vi "湿度测量 - HM1.vi"(7 "CSM Name":string="HM1") -> ()   [LabVIEW 2026, in "UI-湿度测量.lvlib"]
uses:
  Supports/Sample Settings.ctl
  Data ColndSave/Supports/Time and Data.ctl
  <userlib>/_NEVSTOP/Communicable State Machine(CSM)/_Polymophic/CSM - Filter Duplicated Lines.vi
  a3283b4f-3d7d-475f-8286-b95f18be6a9d.vi
  adb26933-f597-44e1-90e5-85e3d61c535a.vi
  c6692627-02fb-4556-9c5d-59e6097d0856.vi
  8c0fc226-3871-4866-9b38-f175316b3ef9.vi
  8417ea6c-3bd9-4cd5-8933-b29b0935beb3.vi
  c0a7cae7-a94b-4088-a6e9-4f476a10c4ba.vi
  <userlib>/_NEVSTOP/Communicable State Machine(CSM)/_Polymophic/CSM - Replace Marks in Messages.vi
  5163a33a-69e0-492d-a74e-a390bdb1a610.vi
  afa19ee1-f3d3-482d-9a92-e9809811bd36.vi
  6c4ca8cd-bc2b-4d91-b813-4304b5b94d16.vi
  <userlib>/_NEVSTOP/Communicable State Machine(CSM)/AdvanceAPI/CSM - Compact Multiple States.vi
  <userlib>/_NEVSTOP/Communicable State Machine(CSM)/AdvanceAPI/CSM - Break Down Multiple States String.vi
  <userlib>/_NEVSTOP/Communicable State Machine(CSM)/_Shared/Remove Comments from Single-line.vi
  <userlib>/_NEVSTOP/Communicable State Machine(CSM)/_Shared/Split Single-line Message.vi
  <userlib>/_NEVSTOP/Communicable State Machine(CSM)/_Shared/Trim Single-line Text.vi
  <userlib>/_NEVSTOP/Communicable State Machine(CSM)/AdvanceAPI/CSM - Revert Arguments-Safe String.vi
  <userlib>/_NEVSTOP/Communicable State Machine(CSM)/AdvanceAPI/CSM - Make String Arguments Safe.vi
  c6692627-02fb-4556-9c5d-59e6097d0856.vi/99de0c97-112a-4c86-9094-c187659127e1.vi
  <userlib>/_NEVSTOP/Communicable State Machine(CSM)/Utility/Build Error Cluster.vi
  8417ea6c-3bd9-4cd5-8933-b29b0935beb3.vi/99de0c97-112a-4c86-9094-c187659127e1.vi
  <userlib>/_NEVSTOP/Communicable State Machine(CSM)/AdvanceAPI/CSM - Keywords.vi
  <userlib>/_NEVSTOP/Communicable State Machine(CSM)/addons/API-String-Arugments-Support/_Support/Data To API String Arguments.vi
  <userlib>/_NEVSTOP/Communicable State Machine(CSM)/addons/INI-Static-Variable-Support/_Support/instances/_CSM - Read File Logger Configuration - v1.0.vi
  <vilib>/Utility/Data Type/Get Type Information.vi
  <userlib>/_NEVSTOP/Communicable State Machine(CSM)/addons/API-String-Arugments-Support/_Support/Data To SingleElementsArray_csm.vi
  <userlib>/_NEVSTOP/Communicable State Machine(CSM)/addons/INI-Static-Variable-Support/_Support/Parse Used Session and Name.vi
  <userlib>/_NEVSTOP/Communicable State Machine(CSM)/addons/INI-Static-Variable-Support/_Support/INI-FGV(lvlibp).vi
  <userlib>/_NEVSTOP/Communicable State Machine(CSM)/addons/INI-Static-Variable-Support/_Support/Populate String with INI Variable.vi
  <userlib>/_NEVSTOP/Communicable State Machine(CSM)/addons/API-String-Arugments-Support/_Support/Convert API String Arguments to Data(variant).vi
  <userlib>/_NEVSTOP/Communicable State Machine(CSM)/addons/API-String-Arugments-Support/_Support/SingleElementsArray To Data_csm.vi
  <userlib>/_NEVSTOP/Communicable State Machine(CSM)/addons/MassData-Parameter/_support/FGV-MassData(lvlibp).vi
  <userlib>/_NEVSTOP/Communicable State Machine(CSM)/Communicable State Machine.lvlib
  Acquisition/Acquisition.lvlib
  <userlib>/_NEVSTOP/Communicable State Machine(CSM)/addons/MassData-Parameter/CSM MassData Parameter Support.lvlib
  <userlib>/_NEVSTOP/Communicable State Machine(CSM)/addons/INI-Static-Variable-Support/INI-Static-Variable-Support.lvlib
  <userlib>/_NEVSTOP/Communicable State Machine(CSM)/addons/Watchdog/CSM Watchdog.lvlib
  <userlib>/_NEVSTOP/Communicable State Machine(CSM)/addons/Logger/CSM File Logger.lvlib
  Logging/Logging.lvlib
  Data ColndSave/Data Collection and Save.lvlib
panel:
  in  "停止":bool
  in  "湿度显示":enum32{"温度采集", "Status"}(tab)
  in  "湿度采集开关":bool
  in  "USB Port":refnum<visa-resource-name>="COM3"
  in  "Interval(s)":dbl=0.5
  out "湿度":waveform(dbl)(graph)
  in  "子程序？":bool
  out "Error Occurred":errorcluster caption="温度采集-错误输出"
  out "State History":string
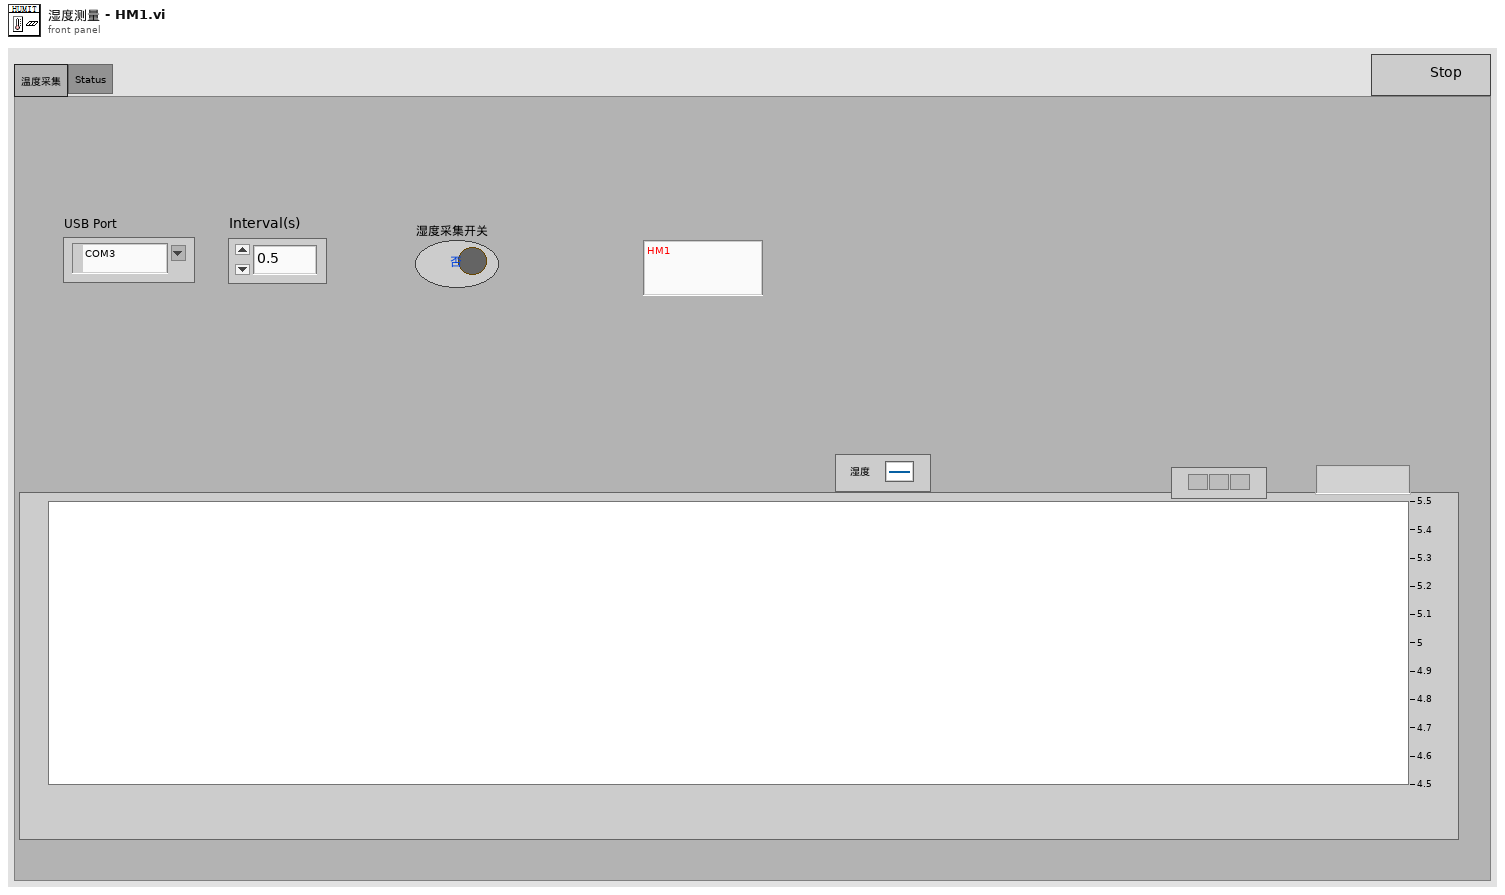
[diagram p1: front panel]
types:
  T1 = cluster{"Enable":bool, "Limit":cluster{"FileSize":i64, "FileNum":i32}, "Timestamp.Format":string, "AutoExit":bool}
  T2 = enum32{"Invalid", "Standard", "Closed", "Hidden", "Minimized", "Maximized"}
  T3 = enum32{"invalid app kind", "Development System", "Run Time System", "Student Edition", "Embedded LabVIEW", "Evaluation", "Custom"}
  T4 = typedef "Communicable State Machine.lvlib/_CSM_Response Source Message.ctl" = cluster{"‘State":string, "’Arguments":string, "’Error":errorcluster}
  T5 = cluster{"Current VI Reference":refnum<vi>, "Close Panel on Exit?":bool}
  T6 = typedef "UI-湿度测量.lvlib/Sample Settings.ctl" = cluster{"USB Port":refnum<visa-resource-name>, "Interval(s)":dbl}
  T7 = typedef "Data Collection and Save.lvlib/Time and Data.ctl" = cluster{"采集时间":timestamp, "Data":dbl[]}
  T8 = cluster{"Core":cluster{"Current VI Reference":refnum<vi>, "Close Panel on Exit?":bool}, "Sample Settings":T6, "Time and Data":T7, "子程序？":bool}
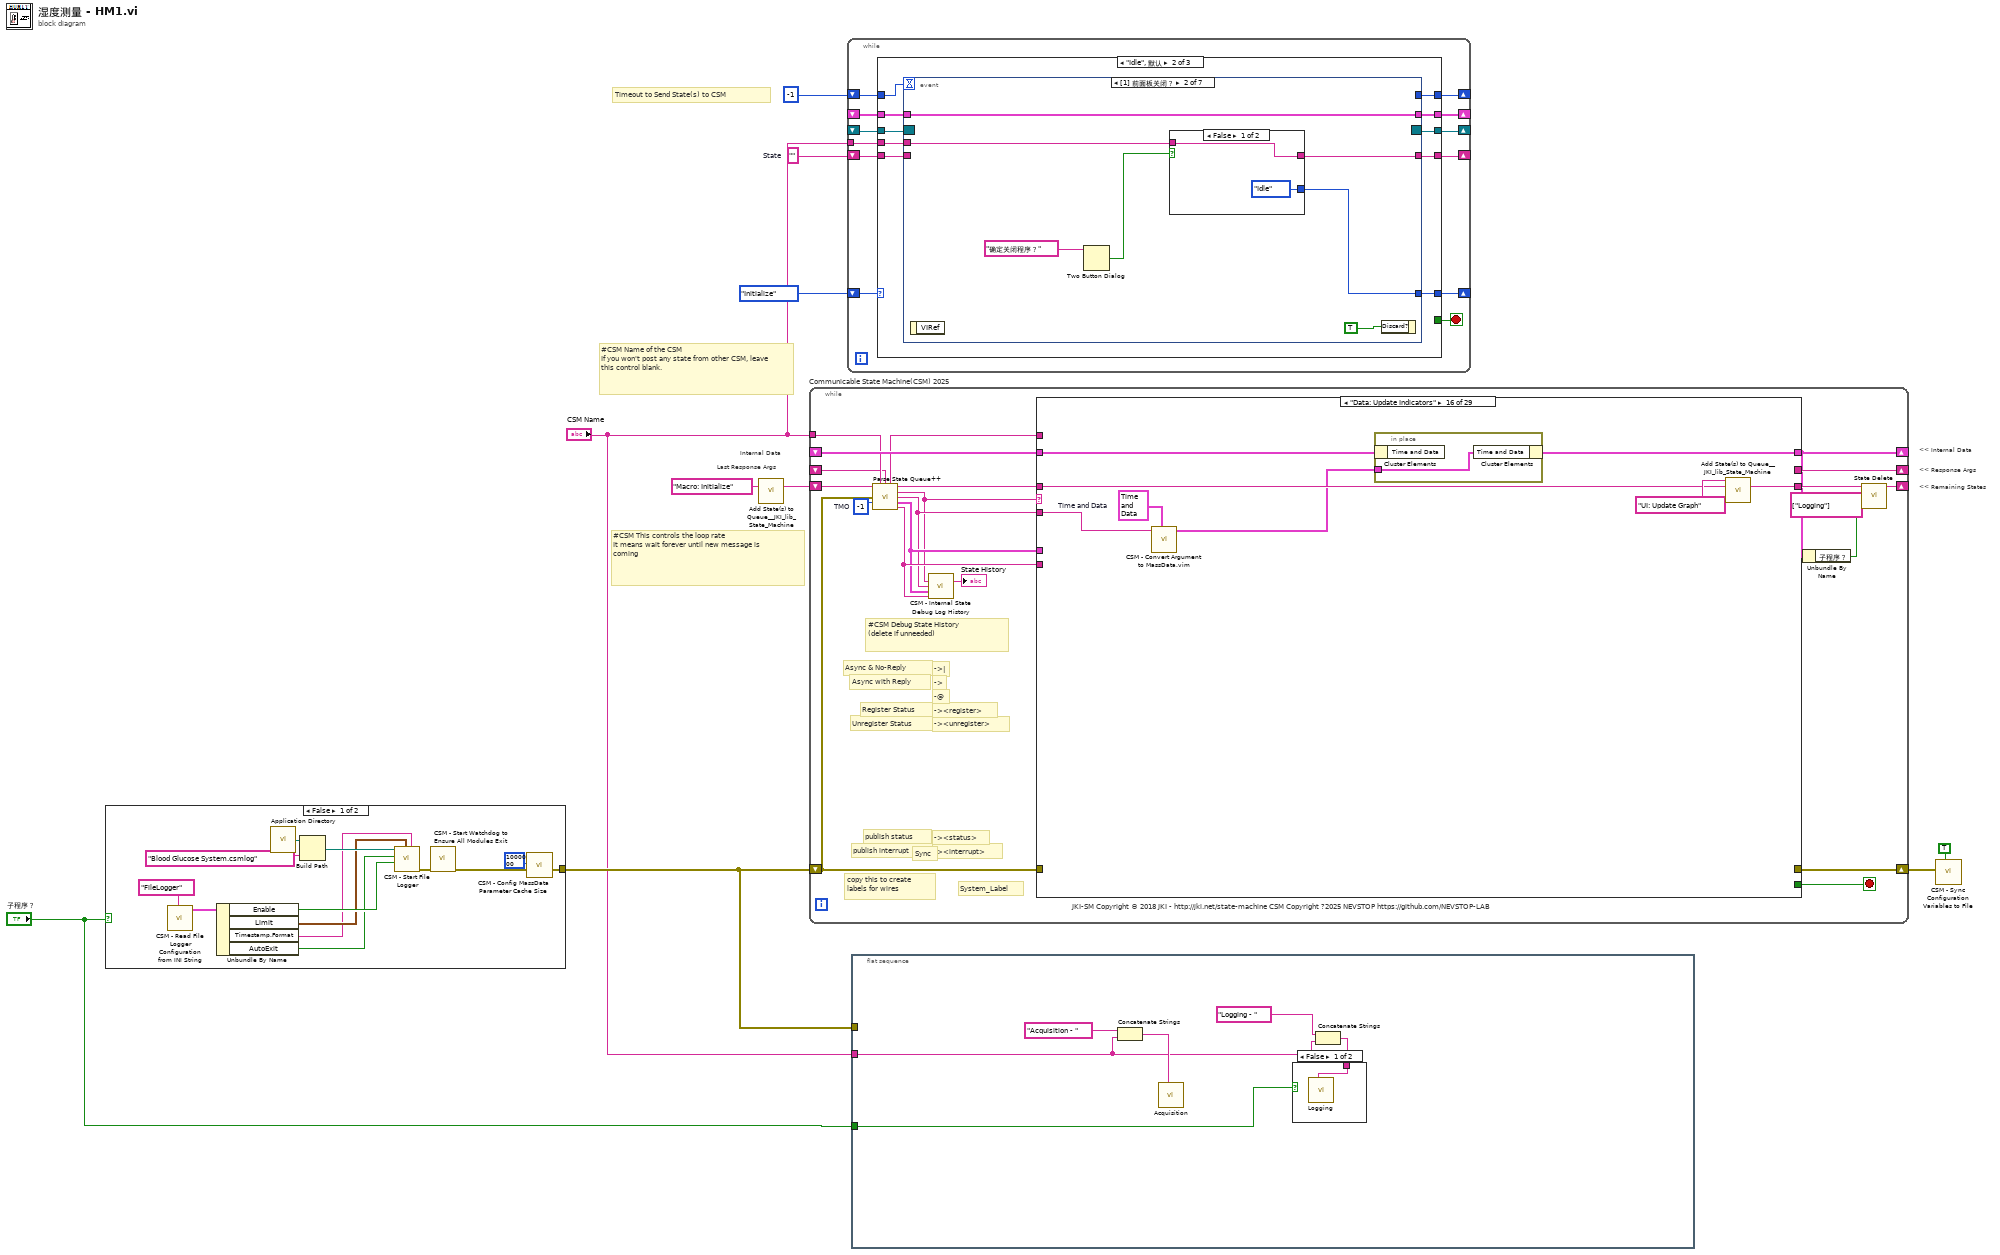
[diagram p0: block diagram]
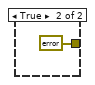
[diagram p2: hidden frame]
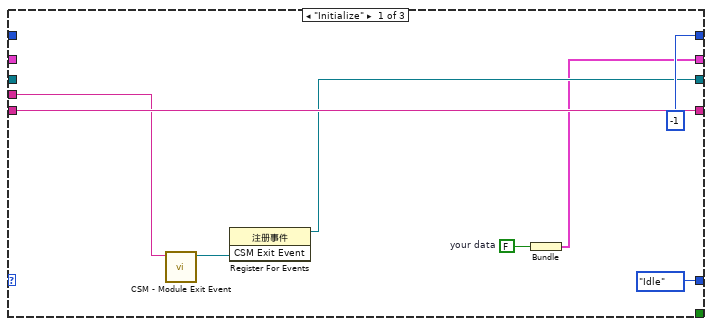
[diagram p4: hidden frame]
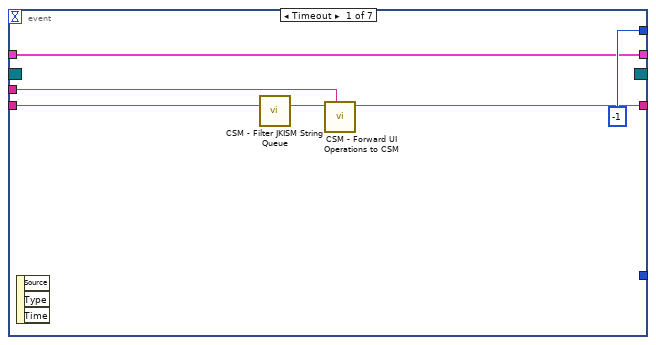
[diagram p5: hidden frame]
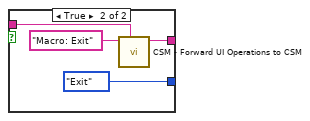
[diagram p6: hidden frame]
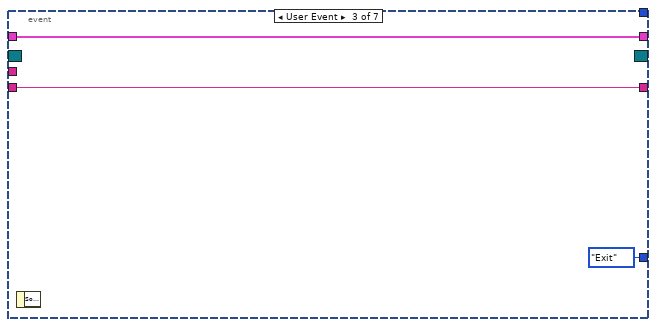
[diagram p7: hidden frame]
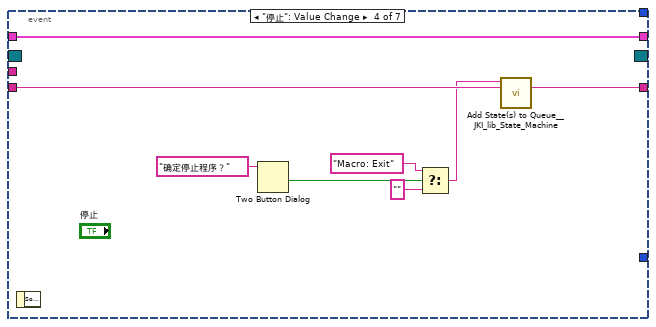
[diagram p8: hidden frame]
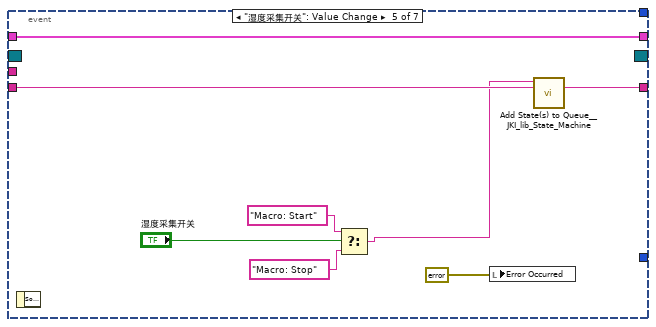
[diagram p9: hidden frame]
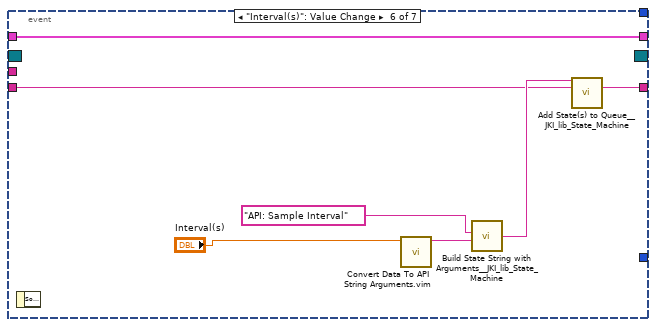
[diagram p10: hidden frame]
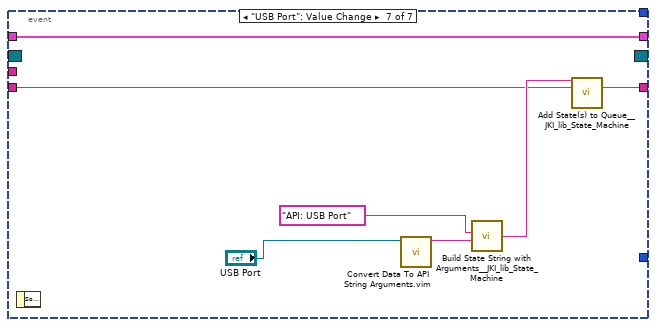
[diagram p11: hidden frame]
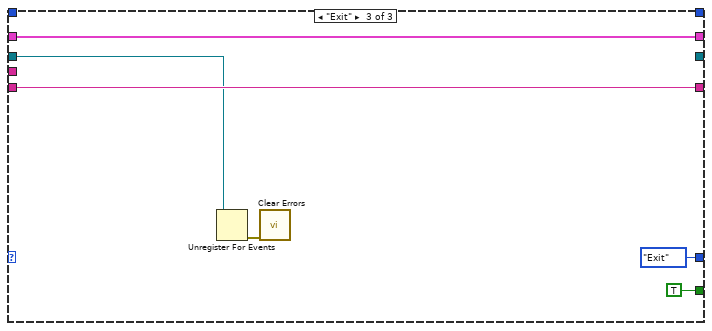
[diagram p12: hidden frame]
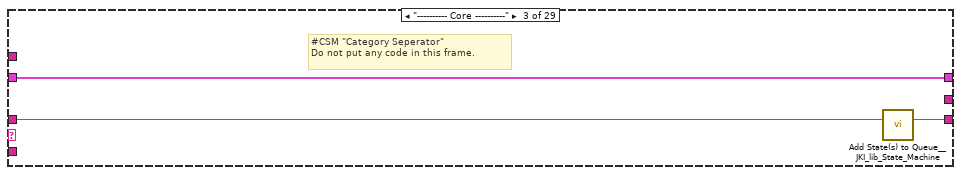
[diagram p15: hidden frame]
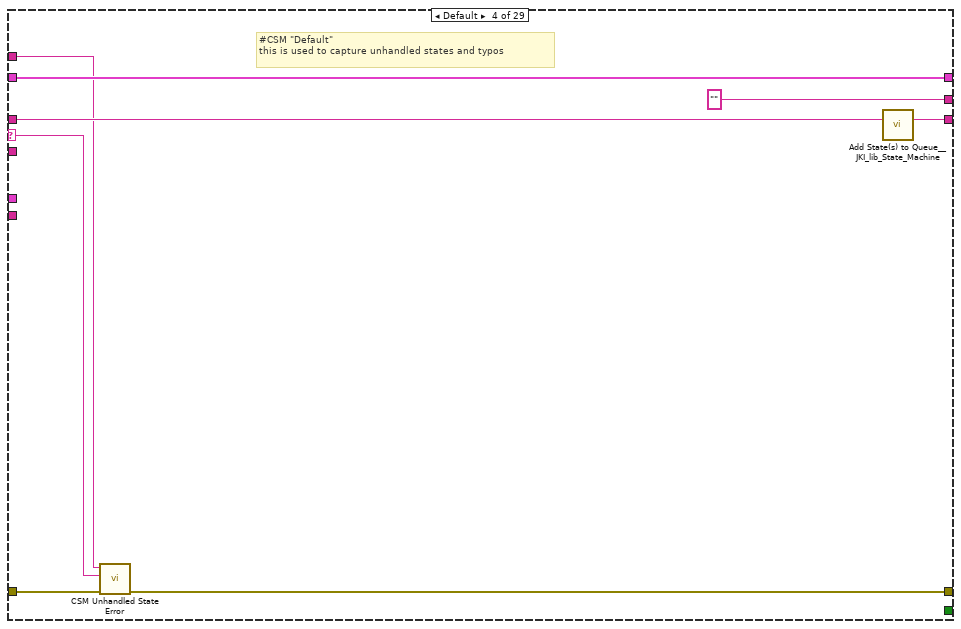
[diagram p16: hidden frame]
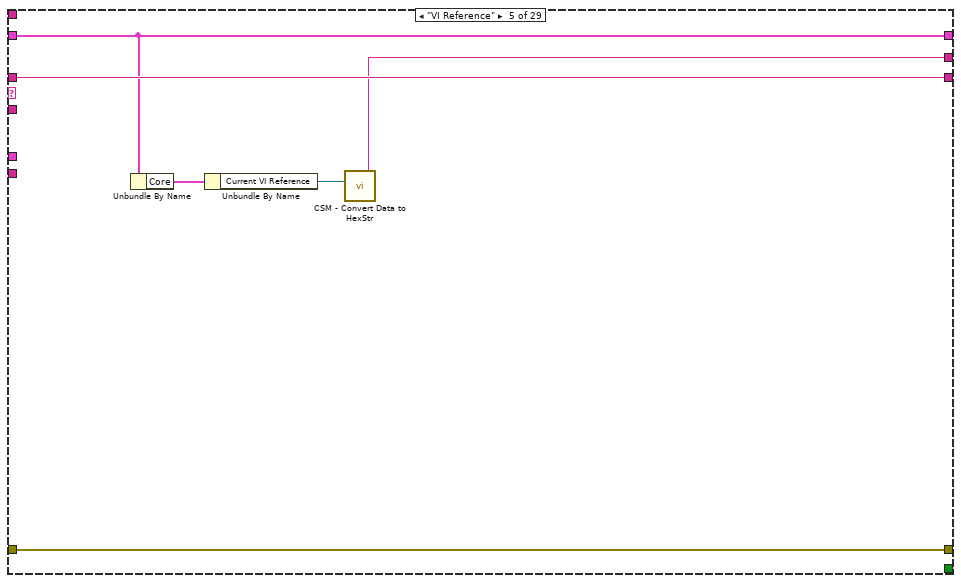
[diagram p17: hidden frame]
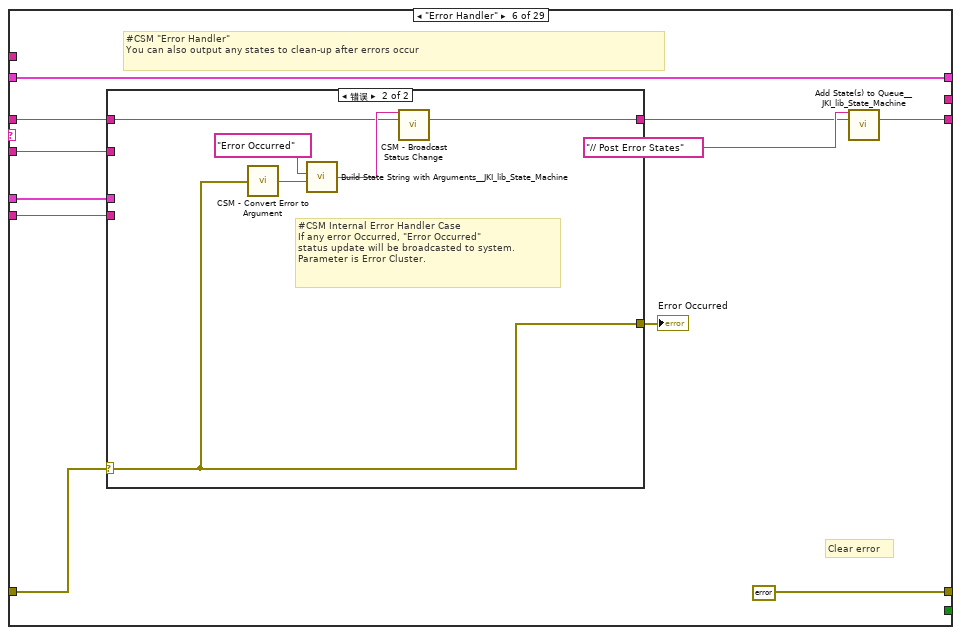
[diagram p18: hidden frame]
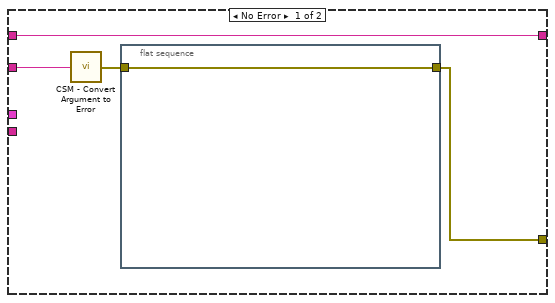
[diagram p19: hidden frame]
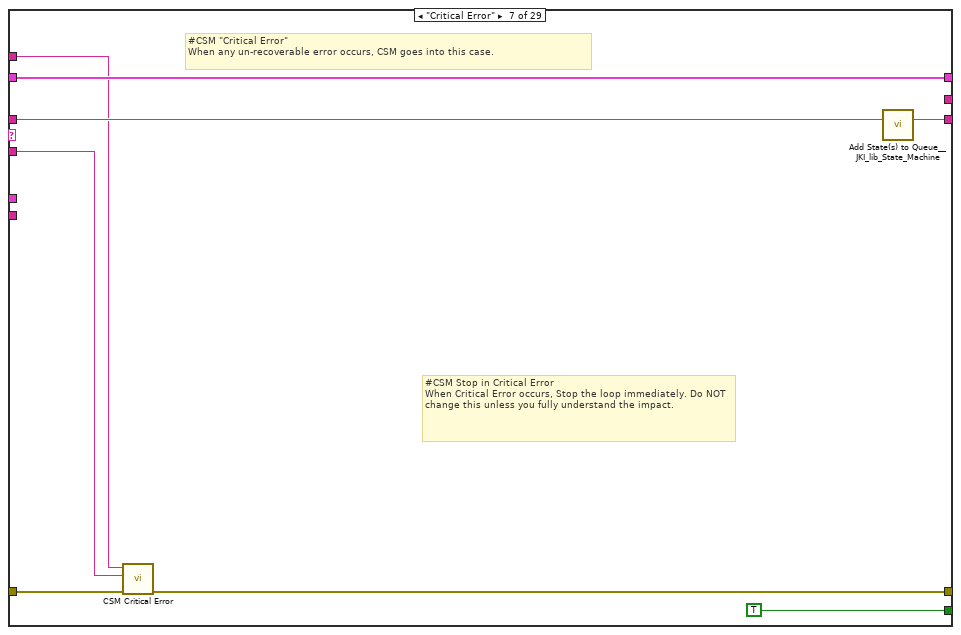
[diagram p20: hidden frame]
diagram:
  w9 = ""  # State
  # "Timeout to Send State(s) to CSM"
  # "Last Response Args"
  # "Internal Data"
  # "#CSM Name of the CSM\nIf you won't post any state from other CSM, leave this control blank."
  # "#CSM This controls the loop rate\nIt means wait forever until new message is coming"
  # "<< Internal Data"
  # "<< Response Args"
  # "<< Remaining States"
  n1 = case shown="False" "子程序？" {
    tunnel: [w11 errorcluster {"status"=FALSE, "code"=0, "source"=""} ("Error out")] -> w5
    frame False {
      n2 = call-poly <userlib>:"CSM - Read File Logger Configuration from INI String.vi"("Section Name(\"FileLogger\")"="FileLogger" ("Section Name(\"\" as Default)")) -> ("FileLogger Configuration-v1"=w18:T1)  [unwired: 7 in, 1 out]
      n3 = Unbundle By Name(w18) -> ("Enable"=w17:bool, "Limit"=w16:cluster{"FileSize":i64, "FileNum":i32}, "Timestamp.Format"=w14:string, "AutoExit"=w15:bool)
      n4 = call <vilib>:"Application Directory.vi"() -> ("Application Directory"=w23:path)
      n5 = Build Path(base path=w23, name or relative path="Blood Glucose System.csmlog") -> (appended path=w21:path)
      n6 = call <userlib>:"CSM - Start File Logger.vi"("Timestamp Format"=w14, "Log Limit"=w16, "Watchdog? (T)"=w17, "Exit When All Module Exist? (F)"=w15, "Log File Path"=w21) -> ("error out"=w20:errorcluster)  [unwired: 4 in, 2 out]
      n7 = call <userlib>:"CSM - Start Watchdog to Ensure All Modules Exit.vi"("error in (no error)"=w20) -> ("error out"=w12:errorcluster)  [unwired: 10 in]
      n8 = call <userlib>:"CSM - Config MassData Parameter Cache Size.vi"("Error in"=w12, "Size (50M)"=1000000 ("size(1M)")) -> ("Error out"=w11:errorcluster)  [unwired: 9 in]
    }
    frame True {
    }
  }
  n9 = call <vilib>:"Add State(s) to Queue__JKI_lib_State_Machine.vi"("State(s) in (\"\")"="Macro: Initialize" ("Init State(\"Macro: Initialize\")")) -> ("States Out"=w6:string)  [unwired: 14 in]
  n10 = while "Communicable State Machine(CSM) 2025" {
    shift-right: [w26] -> _
    shift-left: _ -> [w41]
    shift-right: [w43] -> w3
    shift-left: w5 -> [w31]
    shift-right: [w28] -> _
    shift-left: w6 -> [w44]
    tunnel: "CSM Name" -> [w38]
    shift-right: [w39] -> _
    shift-left: _ -> [w33]
    stop <- w42 stop-if-true
    w40 = -1  # TMO
    # "#CSM Debug State History\n(delete if unneeded)"
    # "-><interrupt>"
    # "-><status>"
    # "-><unregister>"
    # "-><register>"
    # "-@"
    # "->"
    # "->|"
    # "publish interrupt"
    # "publish status"
    # "Unregister Status"
    # "Register Status"
    # "Sync"
    # "Async with Reply"
    # "Async & No-Reply"
    # "JKI-SM Copyright © 2018 JKI - http://jki.net/state-machine CSM Copyright ?2025 NEVSTOP https://github.com/NEVSTOP-LAB"
    # "copy this to create labels for wires"
    # "System_Label"
    n11 = call <userlib>:"Parse State Queue++.vi"("State Queue"=w44, "Name (\"\" to Use UUID)"=w38, "Response Arguments"=w33, "Previous Error"=w31, "Dequeue (1 ms)"=w40) -> ("Name Used"=w32:string, "Remaining States"=w45:string, "Current State"=w34:string, "Arguments"=w35:string, "Additional Information"=w36:T4, "Source CSM"=w37:string)  [unwired: 5 in]
    n12 = call <userlib>:"CSM - Internal State Debug Log History.vi"("State"=w34, "Arguments (\"\")"=w35, ">> Response Source Message >>"=w36, "Source (\"\")"=w37) -> ("Debug Log"=→"State History":string)  [unwired: 11 in]
    n13 = case shown="\"Data: Update Indicators\"" w34 {
      selector: w34 -> [_ _ _ w56 _ _ _ _ _ _ _ _ _ _ _ _ _ _ _ _ _ _ _ _ _ _ _ _ _]
      tunnel: w45 -> [w46 w49 w52 w60 w65 w71 w96 w102 w108 w118 w125 w137 w141 w144 w157 w164 w175 w178 w186 w197 w203 w208 w214 w224 w231 w237 w240 w251 w258]
      tunnel: w35 -> [_ _ _ _ _ w70 w92 w99 w105 w112 _ _ _ _ _ w162 _ _ _ _ w199 _ _ _ _ _ _ w245 w256]
      tunnel: w41 -> [w47 w48 w50 w58 w64 w76 w94 w100 w106 w116 w124 w131 w139 w142 _ w160 w170 w176 w179 w195 w201 w206 w212 w221 w229 w235 w242 w244 w255]
      tunnel: [_ _ _ w53 w66 errorcluster {"status"=FALSE, "code"=0, "source"=""} ("error out") w89 w97 w103 w119 _ _ _ _ _ _ w171 _ _ _ _ _ _ _ _ _ _ _ _] -> w43
      tunnel: w31 -> [_ _ _ w54 w66 w74 w90 w98 w104 _ _ _ _ _ _ _ w172 _ _ _ _ _ _ _ _ _ _ _ _]
      tunnel: [w46 w49 w51 w59 w65 w72 w95 w101 w107 w117 w125 w136 w140 w143 w156 w163 w174 w177 w185 w196 w202 w207 w213 w223 w230 w236 w241 w252 w259] -> w29
      tunnel: [_ _ _ _ _ _ TRUE _ _ _ _ _ TRUE _ _ _ _ _ _ _ _ _ _ _ _ _ _ _ _] -> w42
      tunnel: [w47 w48 w50 w58 w64 w76 w94 w100 w106 w115 w124 w135 w139 w142 w155 w159 w170 w176 w179 w195 w201 w206 w212 w220 w229 w235 w242 w243 w254] -> w26
      tunnel: w37 -> [_ _ _ _ _ w69 _ _ _ w113 _ _ _ _ _ _ _ _ _ _ _ _ _ _ _ _ _ _ _]
      tunnel: w36 -> [_ _ _ _ _ w68 _ _ _ w114 _ _ _ _ _ _ _ _ _ _ _ _ _ _ _ _ _ _ _]
      tunnel: [_ _ _ "" w61 _ _ _ _ _ _ _ _ _ _ _ _ _ _ _ _ _ _ _ _ _ _ _ _] -> w39
      tunnel: w32 -> [_ _ _ w55 _ _ w91 _ _ _ _ _ _ _ w151 _ w167 _ _ _ _ _ w210 w217 w227 w233 _ w249 _]
      frame "", "Idle" {
        # "#CSM \"Idle/Event Handler\"\nexecutes when the state queue is empty"
      }
      frame "CSM Documentation" {
        # "#CSM State Syntax\n\n// Comment line, all text to the right of “//” will be ignored\n// Local Message Example\nDoSth: DoA >> Arguments\n\n// Sync Call Example\nAPI: xxxx >> Arguments -@ TargetModule\n\n// Async Call Example\nAPI: xxxx >> Arguments -> TargetModule\n\n// Async Call without Reply Example\nAPI: xxxx >> Arguments ->| TargetModule\n\n// Broadcast normal status:\nStatus >> StatusArguments  -><status>\n\n// Broadcast Interrupt status:\nInterrupt >> StatusArguments  -><interrupt>\n\n// Register Source Module's status to Handler Module\nStatus@Source Module >> Handler Module@Handler Module -><register>\n\n// Unegister Source Module's status\nStatus@Source Module >> Handler Module -><unregister>"
        # "#CSM README FIRST\n\nCommunicable State Machine(CSM) is a LabVIEW application framework that builds upon JKI State Machine(JKISM). It follows the pattern of JKISM and extends the keywords to describe message communication between modules, including concepts such as Sync-Message, Async-Message, Subscription/Unsubscription of status - essential elements for creating reusable code modules. For more information, please visit the CSM wiki: https://nevstop-lab.github.io/CSM-Wiki/\n\nFor instructions on JKI State Machine, visit: \n    http://jki.net/state-machine/\nFor information about CSM, visit: \n    https://github.com/NEVSTOP-LAB"
        # "#CSM \"Documentation\"\nCase for holding CSM Documenation"
      }
      frame "---------- Core ----------" {
        # "#CSM \"Category Seperator\"\nDo not put any code in this frame."
        n14 = call <vilib>:"Add State(s) to Queue__JKI_lib_State_Machine.vi"("State(s) in (\"\")"=w52) -> ("States Out"=w51:string)  [unwired: 14 in]
      }
      frame Default {
        # "#CSM \"Default\"\nthis is used to capture unhandled states and typos"
        n15 = call <userlib>:"CSM Unhandled State Error.vi"("error in (no error)"=w54, "Undefined State"=w56, "CSM Name"=w55) -> ("error out"=w53:errorcluster)  [unwired: 8 in]
        n16 = call <vilib>:"Add State(s) to Queue__JKI_lib_State_Machine.vi"("State(s) in (\"\")"=w60) -> ("States Out"=w59:string)  [unwired: 14 in]
      }
      frame "VI Reference" {
        n17 = Unbundle By Name(w64) -> ("Core"=w63:T5)
        n18 = Unbundle By Name(w63) -> ("Current VI Reference"=w62:refnum<vi>)
        n19 = call <userlib>:"CSM - Convert Data to HexStr.vi"("Variant"=w62) -> ("HEX String (0-9,A-F)"=w61:string)  [unwired: 8 in]
      }
      frame "Error Handler" {
        # "#CSM \"Error Handler\"\nYou can also output any states to clean-up after errors occur"
        # "Clear error"
        n20 = case shown="错误" w74 {
          selector: w74 -> [_ w83]
          tunnel: [w81 w85] -> w73
          tunnel: w71 -> [w81 w84]
          tunnel: w70 -> [w80 _]
          tunnel: w69 -> [_ _]
          tunnel: w68 -> [_ _]
          tunnel: [w78 w83] -> w67
          frame No Error {
            n21 = call <userlib>:"CSM - Convert Argument to Error.vi"("Argument"=w80) -> ("Error"=w79:errorcluster)  [unwired: 4 in]
            n22 = flat-sequence {
              tunnel: w79 -> [w82]
              tunnel: [w82] -> w78
              frame #0 {
              }
            }
          }
          frame Error {
            # "#CSM Internal Error Handler Case \nIf any error Occurred, \"Error Occurred\" \nstatus update will be broadcasted to system.\nParameter is Error Cluster."
            n23 = call <userlib>:"CSM - Convert Error to Argument.vi"("Error"=w83) -> ("Argument"=w87:string)  [unwired: 4 in]
            n24 = call <vilib>:"Build State String with Arguments__JKI_lib_State_Machine.vi"("Arguments (\"\")"=w87, "State"="Error Occurred" ("Status with Arguments")) -> ("State with Arguments"=w86:string)  [unwired: 4 in]
            n25 = call <userlib>:"CSM - Broadcast Status Change.vi"("Status With Arguments"=w86, "State Queue"=w84) -> ("Remaining States"=w85:string)  [unwired: 13 in]
          }
        }
        "Error Occurred" <- w67
        n26 = call <vilib>:"Add State(s) to Queue__JKI_lib_State_Machine.vi"("State(s) in Front (\"\")"="// Post Error States", "State(s) in (\"\")"=w73) -> ("States Out"=w72:string)  [unwired: 13 in]
      }
      frame "Critical Error" {
        # "#CSM \"Critical Error\"\nWhen any un-recoverable error occurs, CSM goes into this case."
        # "#CSM Stop in Critical Error\nWhen Critical Error occurs, Stop the loop immediately. Do NOT change this unless you fully understand the impact."
        n27 = call <userlib>:"CSM Critical Error.vi"("error in (no error)"=w90, "Arugments (As Reason)"=w92, "CSM Name"=w91) -> ("error out"=w89:errorcluster)  [unwired: 8 in]
        n28 = call <vilib>:"Add State(s) to Queue__JKI_lib_State_Machine.vi"("State(s) in (\"\")"=w96) -> ("States Out"=w95:string)  [unwired: 14 in]
      }
      frame "Target Timeout Error" {
        # "#CSM \"Target Timeout Error\"\nWhen This CSM could not get the sync-call response in time, This CSM goes into this case."
        n29 = call <userlib>:"CSM Target Timeout Error.vi"("error in (no error)"=w98, "Arguments (As CSM Name)"=w99) -> ("error out"=w97:errorcluster)  [unwired: 9 in]
        n30 = call <vilib>:"Add State(s) to Queue__JKI_lib_State_Machine.vi"("State(s) in (\"\")"=w102) -> ("States Out"=w101:string)  [unwired: 14 in]
      }
      frame "Target Error" {
        # "#CSM \"Target Error\"\nWhen This CSM try to communicate with an un-existed CSM, This CSM goes into this case."
        n31 = call <userlib>:"CSM Target Error.vi"("error in (no error)"=w104, "Arguments (As CSM Name)"=w105) -> ("error out"=w103:errorcluster)  [unwired: 9 in]
        n32 = call <vilib>:"Add State(s) to Queue__JKI_lib_State_Machine.vi"("State(s) in (\"\")"=w108) -> ("States Out"=w107:string)  [unwired: 14 in]
      }
      frame "Async Response", "Response" {
        n33 = Unbundle(w114) -> ("‘State"=w111:string, "’Arguments"=w110:string, "’Error"=w109:errorcluster)
        n34 = case shown="默认" w111 {
          tunnel: [w120] -> w117
          tunnel: w118 -> [w121]
          tunnel: [w123] -> w115
          tunnel: w116 -> [w123]
          tunnel: [w122] -> w119
          tunnel: w109 -> [w122]
          tunnel: w113 -> [_]
          tunnel: w112 -> [_]
          tunnel: w110 -> [_]
          frame 默认 {
            # "#CSM \"Async Response\"\nHandle Async-call Response (\"Async Response\" for ->)"
            # "#CSM \"Response\"\nHandle Sync-call Response (\"Response\" for -@)"
            # "#CSM Response Comments\nAfter Message is executed, CSM goes to this state for receive the response.\n    For Async Message(->), \"Async Response\" is used. This CSM will goes to \"Async Message Posted\" immediately and receive the \"Async Response\" after the callee finishes the message.\n    For Sync Message(@),  This CSM will wait until the message is done and immediately goes to \"Response\""
            n35 = call <vilib>:"Add State(s) to Queue__JKI_lib_State_Machine.vi"("State(s) in (\"\")"=w121) -> ("States Out"=w120:string)  [unwired: 14 in]
          }
        }
      }
      frame "Async Message Posted" {
        # "#CSM \"Async Message Posted\"\nAfter Async Message is posted (-> or ->| ), CSM goes to this state for post-action.\nYou can use Argument - State to tell which Async Message is called."
      }
      frame "Initialize Core Data" {
        # "#CSM \"Initialize Core Data\"\nThis is used to determine panel behavior on exit"
        # "originally closed?"
        # "exe?"
        # "If panel starts closed or is an EXE, then close it when we exit"
        n36 = property class="VI"() -> ("FP.State"=w128:T2)  [unwired: 2 in, 2 out]
        n37 = property class="App"() -> ("App.Kind"=w134:T3)  [unwired: 2 in, 2 out]
        n38 = control-ref of="Current VI Reference"() -> (w129:refnum<vi>)
        n39 = Equal?(x=w128, y=T2."Closed" ("Front Panel Window:State")) -> (x = y?=w126:bool)
        n40 = Equal?(x=w134, y=T3."Run Time System" ("Application:Kind")) -> (x = y?=w132:bool)
        n41 = Or(x=w126, y=w132) -> (x .or. y?=w130:bool)
        n42 = Bundle By Name(cluster=w131, "Core.Current VI Reference"=w129, "Core.Close Panel on Exit?"=w130) -> (w135:T8)
        n43 = call <vilib>:"Add State(s) to Queue__JKI_lib_State_Machine.vi"("State(s) in (\"\")"=w137) -> ("States Out"=w136:string)  [unwired: 14 in]
      }
      frame "Exit" {
        # "#CSM \"Exit\"\nCase for exiting the loop. No errors that occur here will be handled."
        n44 = call <vilib>:"Add State(s) to Queue__JKI_lib_State_Machine.vi"("State(s) in (\"\")"=w141) -> ("States Out"=w140:string)  [unwired: 14 in]
      }
      frame "---------- Data ----------" {
        # "#CSM \"Category Seperator\"\nDo not put any code in this frame."
        n45 = call <vilib>:"Add State(s) to Queue__JKI_lib_State_Machine.vi"("State(s) in (\"\")"=w144) -> ("States Out"=w143:string)  [unwired: 14 in]
      }
      frame "Data: Initialize" {
        w150 = T7 {"采集时间"=timestamp(0 s since 1904-01-01), "Data"=[0.0, 0.0]}  # Time and Data
        w147 = T6 {"USB Port"="COM3", "Interval(s)"=0.5}  # Sample Settings
        w154 = T5 {"Current VI Reference"=refnum, "Close Panel on Exit?"=FALSE}  # Core
        # "#CSM \"Data: Initialize\"\nInitialize the shift-register data, here.\n(data names are defined by what you wire into the bundle function)"
        # "#CSM do not delete - used by framework"
        # "#CSM Add new data here."
        # "#CSM Data names and types of shift register data are defined by this bundle."
        n46 = local read "子程序？"() -> (w149:bool)
        n47 = local write "湿度采集开关"(FALSE ("温度采集开关")) -> ()
        n48 = call "CSM - Read Cluster Elements From Session.vim"("Section Name (\"\" as Default)"=w151, "Cluster"=w147) -> ("Cluster out"=w148:T6)  [unwired: 6 in, 1 out]
        n49 = local write "Error Occurred"(errorcluster {"status"=FALSE, "code"=0, "source"=""} ("Error Occurred")) -> ()
        n50 = Select(t=w148, s=TRUE, f=w147) -> (s? t:f=w145:T6)
        n51 = Bundle("Core"=w154, "Sample Settings"=w145, "Time and Data"=w150, "子程序？"=w149) -> (w155:T8)  [unwired: 1 in]
        n52 = call <vilib>:"Add State(s) to Queue__JKI_lib_State_Machine.vi"("State(s) in (\"\")"=w157) -> ("States Out"=w156:string)  [unwired: 14 in]
      }
      frame "Data: Update Indicators" {
        w161 = T7 {"采集时间"=timestamp(0 s since 1904-01-01), "Data"=[]}  # Time and Data
        n53 = call "CSM - Convert Argument to MassData.vim"("Type"=w161, "MassData Argument"=w162) -> ("Data"=w158:T7)  [unwired: 6 in, 1 out]
        n54 = in-place {
          in-place-border: w158 -> [w166]
          n55 = in-place-cluster #1(w160) -> ()  [unwired: 1 out]
          n56 = in-place-cluster #1("Time and Data"=w166) -> (w159:T8)
        }
        n57 = call <vilib>:"Add State(s) to Queue__JKI_lib_State_Machine.vi"("State(s) in Front (\"\")"="UI: Update Graph" ("State(s) in Front (\"\")"), "State(s) in (\"\")"=w164) -> ("States Out"=w163:string)  [unwired: 13 in]
      }
      frame "Data: Cleanup" {
        # "#CSM \"Data: Cleanup\"\nCleanup any data and references, here.\n(this is called automatically, by the Macro: Exit)"
        n58 = Unbundle By Name(w170) -> ("Core.Current VI Reference"=w173:refnum<vi>, "Sample Settings"=w168:T6)
        n59 = call "CSM - Write Configuration Variable.vim"("Section Name (\"\" as Default)"=w167, "Configuration"=w168) -> ()  [unwired: 6 in, 2 out]
        n60 = Close Reference(reference=w173, error in (no error)=w172) -> (error out=w171:errorcluster)
        n61 = local write "湿度采集开关"(FALSE ("温度采集开关")) -> ()
        n62 = call <vilib>:"Add State(s) to Queue__JKI_lib_State_Machine.vi"("State(s) in (\"\")"=w175) -> ("States Out"=w174:string)  [unwired: 14 in]
      }
      frame "---------- UI ----------" {
        # "#CSM \"Category Seperator\"\nDo not put any code in this frame."
        n63 = call <vilib>:"Add State(s) to Queue__JKI_lib_State_Machine.vi"("State(s) in (\"\")"=w178) -> ("States Out"=w177:string)  [unwired: 14 in]
      }
      frame "UI: Initialize" {
        # "#CSM \"Category Seperator\"\nDo not put any code in this frame."
        n64 = Unbundle By Name(w179) -> ("Sample Settings.USB Port"=w183:refnum<visa-resource-name>, "Sample Settings.Interval(s)"=w182:dbl, "子程序？"=w181:bool)
        n65 = Not(x=w181) -> (.not. x?=w184:bool)
        n66 = local write "USB Port"(w183) -> ()
        n67 = local write "Interval(s)"(w182) -> ()
        n68 = property on="停止" class="Bool"("Visible"=w184) -> ()  [unwired: 2 in, 2 out]
        n69 = property on="湿度" class="WFChart (严格)"("History Data"=waveform(dbl)[] [] ("历史数据")) -> ()  [unwired: 2 in, 2 out]
        n70 = call <vilib>:"Add State(s) to Queue__JKI_lib_State_Machine.vi"("State(s) in (\"\")"=w186) -> ("States Out"=w185:string)  [unwired: 14 in]
      }
      frame "UI: Update Graph" {
        # "#CSM \"Category Seperator\"\nDo not put any code in this frame."
        n71 = Unbundle By Name(w195) -> ("Time and Data.Data"=w192:dbl[], "Sample Settings.Interval(s)"=w189:dbl, "Time and Data.采集时间"=w190:timestamp)
        n72 = Index Array(array=w192) -> (element #1=w191:dbl, element #2=w188:dbl)  [unwired: 2 in]
        n73 = Build Array(w191) -> (w194:dbl[])
        n74 = Build Array(w188) -> (w193:dbl[])
        n75 = Bundle By Name("Y"=w194, "t0"=w190, "dt"=w189) -> ()  [unwired: 1 in, 1 out]
        n76 = Bundle By Name("Y"=w193, "t0"=w190, "dt"=w189) -> (→"湿度":waveform(dbl))  [unwired: 1 in]
        n77 = call <vilib>:"Add State(s) to Queue__JKI_lib_State_Machine.vi"("State(s) in (\"\")"=w197) -> ("States Out"=w196:string)  [unwired: 14 in]
      }
      frame "UI: Auto Zoom" {
        # "#CSM \"Category Seperator\"\nDo not put any code in this frame."
        n78 = call "Convert API String Arguments to Data.vim"("Reference Type"=FALSE ("Chart Auto Zoom"), "API String"=w199) -> ("Data"=w198:bool)  [unwired: 6 in, 1 out]
        n79 = case shown="False" w198 {
          tunnel: [u8 0 ("X标尺.标尺调节") u8 2 ("X标尺.标尺调节")] -> _
          frame False {
          }
          frame True {
          }
        }
        n80 = call <vilib>:"Add State(s) to Queue__JKI_lib_State_Machine.vi"("State(s) in (\"\")"=w203) -> ("States Out"=w202:string)  [unwired: 14 in]
      }
      frame "---------- Macro ----------" {
        # "#CSM \"Category Seperator\"\nDo not put any code in this frame."
        n81 = call <vilib>:"Add State(s) to Queue__JKI_lib_State_Machine.vi"("State(s) in (\"\")"=w208) -> ("States Out"=w207:string)  [unwired: 14 in]
      }
      frame "Macro: Initialize" {
        w211 = "Data: Initialize\nInitialize Core Data\nUI: Initialize\n\n//Permanent registrations\nAcquired Data@Acquisition - <1> >> Data: Update Indicators -><register>\nAcquired Data@Acquisition - <1> >> API: Log@Logging - <1> -><register>\n\n//Error registrations\nError Occurred@Acquisition - <1> >> Error Handler -><register>\nError Occurred@Logging - <1> >> Error Handler -><register>\n\n//Dynamic registrations\n// 订阅/取消订阅\n//Status@SourceModule >> API@TargetModule -><register as interrupt>\n//UrgentEvent @SourceModule >> API@TargetModule -><register as status>\n\n\n\n//Launch Acquisition Module\n"  # Data: Initialize Initialize Core Data UI: Initialize  //Permanent registrations Acquired Data@Acquisition - <1> >> Data: Update Indicators -><register> Acquired Data@Acquisition - <1> >> API: Log@Logging - <1> -><register>  //Error registrations Error Occurred@Acquisition - <1> >> Error Handler -><register> Error Occurred@Logging - <1> >> Error Handler -><register>  //Dynamic registrations // 订阅/取消订阅 //Status@SourceModule >> API@TargetModule -><register as interrupt> //UrgentEvent @SourceModule >> API@TargetModule -><register as status>    //Launch Acquisition Module
        # "#CSM \"Macro: Initialize\"\nInitialization Macro (This is called once, when the VI starts)"
        n82 = call-poly <userlib>:"Build Message with Arguments++.vi"("States With Replace Token"=w211, "<1>"=w210) -> ("States"=w209:string)  [unwired: 13 in]
        n83 = call <vilib>:"Add State(s) to Queue__JKI_lib_State_Machine.vi"("State(s) in Front (\"\")"=w209, "State(s) in (\"\")"=w214) -> ("States Out"=w213:string)  [unwired: 13 in]
      }
      frame "Macro: Start" {
        n84 = Unbundle By Name(w221) -> ("Sample Settings"=w222:T6)
        n85 = local write "湿度采集开关"(TRUE ("温度采集开关")) -> ()
        n86 = call "Convert Data To API String Arguments.vim"("Data"=w222) -> ("API String"=w218:string)  [unwired: 7 in, 1 out]
        n87 = call-poly <userlib>:"Build Message with Arguments++.vi"("States With Replace Token"="API: Start >> <param> -@ Acquisition - <1>\nAPI: Start  -@ Logging - <1>" ("State"), "<param>"=w218, "<1>"=w217) -> ("States"=w215:string)  [unwired: 12 in]
        n88 = Bundle By Name(cluster=w221, "Sample Settings"=w222) -> (w220:T8)
        n89 = call <vilib>:"Add State(s) to Queue__JKI_lib_State_Machine.vi"("State(s) in Front (\"\")"=w215, "State(s) in (\"\")"=w224) -> ("States Out"=w223:string)  [unwired: 13 in]
      }
      frame "Macro: Stop" {
        # "#CSM \"Macro: Exit\"\nExit Macro (This is called once, when the VI exits)"
        n90 = local write "湿度采集开关"(FALSE ("温度采集开关")) -> ()
        n91 = call-poly <userlib>:"Build Message with Arguments++.vi"("States With Replace Token"="//Send Message to Other CSM Modules\nAPI: Stop -@ Acquisition - <1>\nAPI: Stop -@ Logging - <1>", "<1>"=w227) -> ("States"=w225:string)  [unwired: 13 in]
        n92 = call <vilib>:"Add State(s) to Queue__JKI_lib_State_Machine.vi"("State(s) in Front (\"\")"=w225, "State(s) in (\"\")"=w231) -> ("States Out"=w230:string)  [unwired: 13 in]
      }
      frame "Macro: Exit" {
        w234 = "//Exit\nMacro: Exit-@Acquisition - <1>\nMacro: Exit-@Logging - <1>\n\n//Permanent unregistrations\nAcquired Data@Acquisition - <1> >> Data: Update Indicators -><unregister>\nAcquired Data@Acquisition - <1> >> API: Log@Logging - <1> -><unregister>\n\n//Permanent unregistrations\nError Occurred@Acquisition - <1> >> Error Handler -><unregister>\nError Occurred@Logging - <1> >> Error Handler -><unregister>\n\nData: Cleanup\nExit"  # //Exit Macro: Exit-@Acquisition - <1> Macro: Exit-@Logging - <1>  //Permanent unregistrations Acquired Data@Acquisition - <1> >> Data: Update Indicators -><unregister> Acquired Data@Acquisition - <1> >> API: Log@Logging - <1> -><unregister>  //Permanent unregistrations Error Occurred@Acquisition - <1> >> Error Handler -><unregister> Error Occurred@Logging - <1> >> Error Handler -><unregister>  Data: Cleanup Exit
        # "#CSM \"Macro: Exit\"\nExit Macro (This is called once, when the VI exits)"
        n93 = disable-structure shown="禁用" {
          frame Disabled {
            # "#NOTE\nHelper VI is equivalent to other case"
            n94 = call <userlib>:"CSM - Build Exit Messages of CSMs.vi"("State With Arguments (\"Macro: Exit“)"="Macro: Exit" ("State with Arguments(\"Macro: Exit“)"), "CSMs"=string[] ["AcquisitionTP1", "//LoggingTP1"]) -> ()  [unwired: 13 in, 1 out]
          }
          frame Enabled {
          }
        }
        n95 = call-poly <userlib>:"Build Message with Arguments++.vi"("States With Replace Token"=w234, "<1>"=w233) -> ("States"=w232:string)  [unwired: 13 in]
        n96 = call <vilib>:"Add State(s) to Queue__JKI_lib_State_Machine.vi"("State(s) in Front (\"\")"=w232, "State(s) in (\"\")"=w237) -> ("States Out"=w236:string)  [unwired: 13 in]
      }
      frame "---------- API ----------" {
        # "#CSM \"Category Seperator\"\nDo not put any code in this frame."
        n97 = call <vilib>:"Add State(s) to Queue__JKI_lib_State_Machine.vi"("State(s) in (\"\")"=w240) -> ("States Out"=w241:string)  [unwired: 14 in]
      }
      frame "API: Sample Interval" {
        # "#CSM \"Category Seperator\"\nDo not put any code in this frame."
        n98 = call "Convert API String Arguments to Data.vim"("Reference Type"=0.5 ("Interval(s)"), "API String"=w245) -> ("Data"=w246:dbl)  [unwired: 6 in, 1 out]
        n99 = call-poly <userlib>:"Build Message with Arguments++.vi"("States With Replace Token"="API: Sample Interval >> <param> ->| Acquisition - <1>" ("State"), "<param>"=w245, "<1>"=w249) -> ("States"=w248:string)  [unwired: 12 in]
        n100 = call <vilib>:"Add State(s) to Queue__JKI_lib_State_Machine.vi"("State(s) in Front (\"\")"=w248, "State(s) in (\"\")"=w251) -> ("States Out"=w252:string)  [unwired: 13 in]
        n101 = Bundle By Name(cluster=w244, "Sample Settings.Interval(s)"=w246) -> (w243:T8)
      }
      frame "API: USB Port" {
        # "#CSM \"Category Seperator\"\nDo not put any code in this frame."
        n102 = call "Convert API String Arguments to Data.vim"("Reference Type"=refnum<visa-resource-name> "COM3" ("USB Port"), "API String"=w256) -> ("Data"=w257:refnum<visa-resource-name>)  [unwired: 6 in, 1 out]
        n103 = call <vilib>:"Add State(s) to Queue__JKI_lib_State_Machine.vi"("State(s) in (\"\")"=w258) -> ("States Out"=w259:string)  [unwired: 14 in]
        n104 = Bundle By Name(cluster=w255, "Sample Settings.USB Port"=w257) -> (w254:T8)
      }
    }
    n105 = Unbundle By Name(w26) -> ("子程序？"=w25:bool)
    n106 = call "State Delete.vi"("Delete?(F)"=w25, "CSM name to delete"=string[] ["Logging"], "State In"=w29) -> ("State Out"=w28:string)  [unwired: 8 in]
  }
  n107 = while {
    shift-right: [w270] -> _
    shift-left: enum16{"Idle", "Initialize", "Exit"}."Initialize" -> [w271]
    tunnel: "CSM Name" -> [w268]
    shift-right: [w266] -> _
    shift-left: w9 -> [w267]
    shift-right: [w264] -> _
    shift-left: -1 -> [w265]
    shift-right: [w263] -> _
    shift-left: _ -> [w262]
    shift-right: [w261] -> _
    shift-left: _ -> [w260]
    stop <- w269 stop-if-true
    n108 = case shown="\"Idle\", 默认" w271 {
      tunnel: [enum16{"Idle", "Initialize", "Exit"}."Idle" w289 enum16{"Idle", "Initialize", "Exit"}."Exit"] -> w270
      tunnel: [_ _ TRUE] -> w269
      tunnel: w268 -> [w275 w288 _]
      tunnel: w267 -> [w278 w286 w345]
      tunnel: [w278 w287 w345] -> w266
      tunnel: w265 -> [_ w284 _]
      tunnel: [-1 w285 _] -> w264
      tunnel: [w274 w282 _] -> w263
      tunnel: w262 -> [_ w283 w344]
      tunnel: [w272 w280 w342] -> w261
      tunnel: w260 -> [_ w281 w342]
      frame "Initialize" {
        w273 = FALSE  # your data
        n109 = call <userlib>:"CSM - Module Exit Event.vi"("Name (\"\" to Use UUID) In"=w275) -> ("CSM Exit Event"=w276:refnum<user-event>)  [unwired: 8 in, 2 out]
        n110 = register-events(w276) -> (reference out=w274:refnum<event-registration>)  [unwired: 2 in, 1 out]
        n111 = Bundle("your data"=w273) -> (w272:cluster{"your data":bool})  [unwired: 1 in]
      }
      frame "Idle", Default {
        n112 = event shown="[1] 前面板关闭？" {
          selector: w283 -> [_ _ _ _ _ _ _]
          dyn-events: [_ _ _ _ _ _ _] -> w282
          timeout: w284 -> [_ _ _ _ _ _ _]
          tunnel: [_ w296 enum16{"Idle", "Initialize", "Exit"}."Exit" _ _ _ _] -> w289
          tunnel: w288 -> [w291 w301 _ _ _ _ _]
          tunnel: w286 -> [w294 _ w311 w317 w326 w330 w337]
          tunnel: [w292 w300 w311 w318 w325 w329 w336] -> w287
          tunnel: [-1 _ _ _ _ _ _] -> w285
          tunnel: w281 -> [w290 w299 w309 w319 w327 w334 w341]
          tunnel: [w290 w299 w309 w319 w327 w334 w341] -> w280
          event Timeout {
            n113 = event-data() -> ()  [unwired: 1 in, 3 out]
            n114 = call-poly <userlib>:"CSM - Filter JKISM String Queue.vi"("States In"=w294) -> ("States Out"=w293:string)  [unwired: 14 in]
            n115 = call <userlib>:"CSM - Forward UI Operations to CSM.vi"("Name (\"\" to Use UUID)"=w291, "State(s) In (\"\")"=w293) -> ("States Out"=w292:string)  [unwired: 8 in, 1 out]
          }
          event Panel Close? {
            n116 = event-data() -> ()  [unwired: 1 in, 1 out]
            n117 = Two Button Dialog(message="确定关闭程序？" ("消息")) -> (T button?=w297:bool)  [unwired: 2 in]
            n118 = case shown="False" w297 {
              tunnel: w301 -> [w304 w307]
              tunnel: [w304 w306] -> w300
              tunnel: [enum16{"Idle", "Initialize", "Exit"}."Idle" enum16{"Idle", "Initialize", "Exit"}."Exit"] -> w296
              frame False {
              }
              frame True {
                n119 = call <userlib>:"CSM - Forward UI Operations to CSM.vi"("Name (\"\" to Use UUID)"=w307, "State(s) In (\"\")"="Macro: Exit" ("State")) -> ("States Out"=w306:string)  [unwired: 8 in, 1 out]
              }
            }
            n120 = event-data("Discard?"=TRUE) -> ()  [unwired: 1 in, 1 out]
          }
          event User Event {
            n121 = event-data() -> ()  [unwired: 1 in, 1 out]
          }
          event "停止": Value Change {
            n122 = event-data() -> ()  [unwired: 1 in, 1 out]
            n123 = Two Button Dialog(message="确定停止程序？" ("消息")) -> (T button?=w314:bool)  [unwired: 2 in]
            n124 = Select(t="Macro: Exit" ("State(s) in Front (\"\")"), s=w314, f="") -> (s? t:f=w312:string)
            n125 = call <vilib>:"Add State(s) to Queue__JKI_lib_State_Machine.vi"("State(s) in Front (\"\")"=w312, "State(s) in (\"\")"=w317) -> ("States Out"=w318:string)  [unwired: 13 in]
          }
          event "湿度采集开关": Value Change {
            n126 = event-data() -> ()  [unwired: 1 in, 1 out]
            n127 = Select(t="Macro: Start" ("State(s) in Front (\"\")"), s="湿度采集开关", f="Macro: Stop" ("State(s) in Front (\"\")")) -> (s? t:f=w321:string)
            n128 = local write "Error Occurred"(errorcluster {"status"=FALSE, "code"=0, "source"=""} ("错误常量")) -> ()
            n129 = call <vilib>:"Add State(s) to Queue__JKI_lib_State_Machine.vi"("State(s) in Front (\"\")"=w321, "State(s) in (\"\")"=w326) -> ("States Out"=w325:string)  [unwired: 13 in]
          }
          event "Interval(s)": Value Change {
            n130 = event-data() -> ()  [unwired: 1 in, 1 out]
            n131 = call "Convert Data To API String Arguments.vim"("Data"="Interval(s)") -> ("API String"=w332:string)  [unwired: 7 in, 1 out]
            n132 = call <vilib>:"Build State String with Arguments__JKI_lib_State_Machine.vi"("Arguments (\"\")"=w332, "State"="API: Sample Interval" ("State(s) in Front (\"\")")) -> ("State with Arguments"=w331:string)  [unwired: 4 in]
            n133 = call <vilib>:"Add State(s) to Queue__JKI_lib_State_Machine.vi"("State(s) in Front (\"\")"=w331, "State(s) in (\"\")"=w330) -> ("States Out"=w329:string)  [unwired: 13 in]
          }
          event "USB Port": Value Change {
            n134 = event-data() -> ()  [unwired: 1 in, 1 out]
            n135 = call "Convert Data To API String Arguments.vim"("Data"="USB Port") -> ("API String"=w339:string)  [unwired: 7 in, 1 out]
            n136 = call <vilib>:"Build State String with Arguments__JKI_lib_State_Machine.vi"("Arguments (\"\")"=w339, "State"="API: USB Port" ("State(s) in Front (\"\")")) -> ("State with Arguments"=w338:string)  [unwired: 4 in]
            n137 = call <vilib>:"Add State(s) to Queue__JKI_lib_State_Machine.vi"("State(s) in Front (\"\")"=w338, "State(s) in (\"\")"=w337) -> ("States Out"=w336:string)  [unwired: 13 in]
          }
        }
      }
      frame "Exit" {
        n138 = Unregister For Events(event registration refnum=w344) -> (error out=w343:errorcluster)  [unwired: 1 in]
        n139 = call <vilib>:"Clear Errors.vi"("error in (no error)"=w343) -> ()  [unwired: 5 in, 2 out]
      }
    }
  }
  n140 = flat-sequence {
    tunnel: w5 -> [_]
    tunnel: "CSM Name" -> [w350]
    tunnel: "子程序？" -> [w348]
    frame #0 {
      n141 = Concatenate Strings("Acquisition - " ("Name(\"\" to use uuid)"), w350) -> (w352:string)
      n142 = call "Acquisition.vi"("CSM Name"=w352) -> ()  [unwired: 11 in]
      n143 = Concatenate Strings("Logging - " ("Name(\"\" to use uuid)"), w350) -> (w349:string)
      n144 = case shown="False" w348 {
        tunnel: w349 -> [w354 _]
        frame False {
          n145 = call "Logging.vi"("CSM Name"=w354) -> ()  [unwired: 11 in]
        }
        frame True {
        }
      }
    }
  }
  n146 = call <userlib>:"CSM - Sync Configuration Variables to File.vi"("All Temp Variable to Default Ini(F)"=TRUE, "error in (no error)"=w3) -> ()  [unwired: 7 in, 1 out]
